vi "conf FCC Main RSE Measurement.vi"(8 "error in (no error)":errorcluster, 11 "SA Measurement in":refnum<class "SA Measurement.lvclass">) -> (0 "error out":errorcluster, 3 "SA Measurement out":refnum<class "SA Measurement.lvclass">)   [LabVIEW 2023, in "Spectrum Analyzer.lvlib" / "SA Measurement.lvclass"]
uses:
  SA Measurement.lvclass
  TYPE DEFINITION/TYPE RBW and VBW Select.ctl
  TYPE DEFINITION/Keysight 9020A/TYPE Measurement Preset.ctl
  SA Measurement.lvclass/SA Measurement.ctl
  Interface_Spectrum/Interface_Spectrum.lvclass
  Spectrum Analyzer.lvlib
  TYPE DEFINITION/TYPE Average Mode Select.ctl
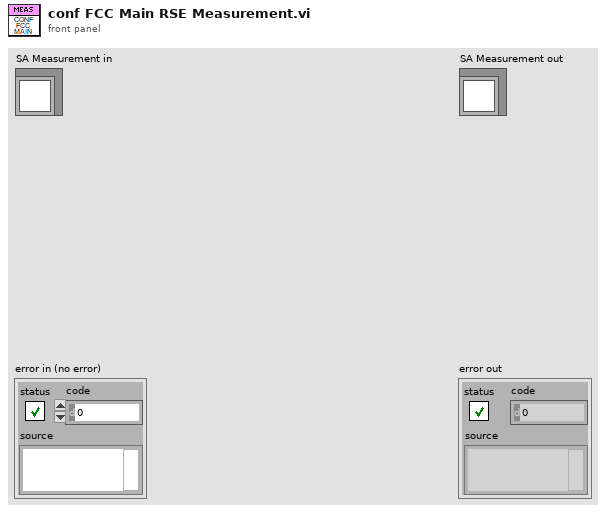
[diagram p1: front panel]
types:
  T1 = typedef "Spectrum Analyzer.lvlib/TYPE Average Mode Select.ctl" = enum16{"Linear(Voltage Avg)", "Video(Log)", "Power"}
  T2 = typedef "Spectrum Analyzer.lvlib/TYPE Measurement Preset.ctl" = enum16{"Sweep SA Mode", "Channel Power", "Occupied BW", "ACP", "Spurious Emission", "Spurious Emission Mask", "Burst Power (Transmit Power)"}
  T3 = typedef "Spectrum Analyzer.lvlib/TYPE RBW and VBW Select.ctl" = enum16{"Res BW", "Video BW"}
  T4 = typedef "Spectrum Analyzer.lvlib/TYPE Y-axis Unit.ctl" = enum16{"dBm", "dBmV", "dBuV", "dBpW", "Volt", "Ampere", "Watt"}
  T5 = typedef "Spectrum Analyzer.lvlib/TYPE Start and Stop Frequency.ctl" = cluster{"Start":dbl, "Stop":dbl}
  T6 = typedef "Spectrum Analyzer.lvlib/TYPE Reference Level and Atten Param.ctl" = cluster{"Reference Level":dbl, "Atten":i32, "Atten Auto?":bool, "Reference Level Offset":dbl}
  T7 = typedef "Spectrum Analyzer.lvlib/TYPE Display Trace Mode Select.ctl" = enum16{"Clear Write", "Max Hold", "Min Hold", "Average", "View"}
  T8 = typedef "Spectrum Analyzer.lvlib/TYPE Detect Mode Select.ctl" = enum16{"Det Auto (Normal)", "Auto Peak", "Positive Peak", "Negative Peak", "Sample", "RMS", "Average", "Quasipeak", "CISPR Average", "RMS Average"}
  T9 = cluster{"Trace Mode":T7, "Detector Type":T8, "Detect Auto?":bool}[]
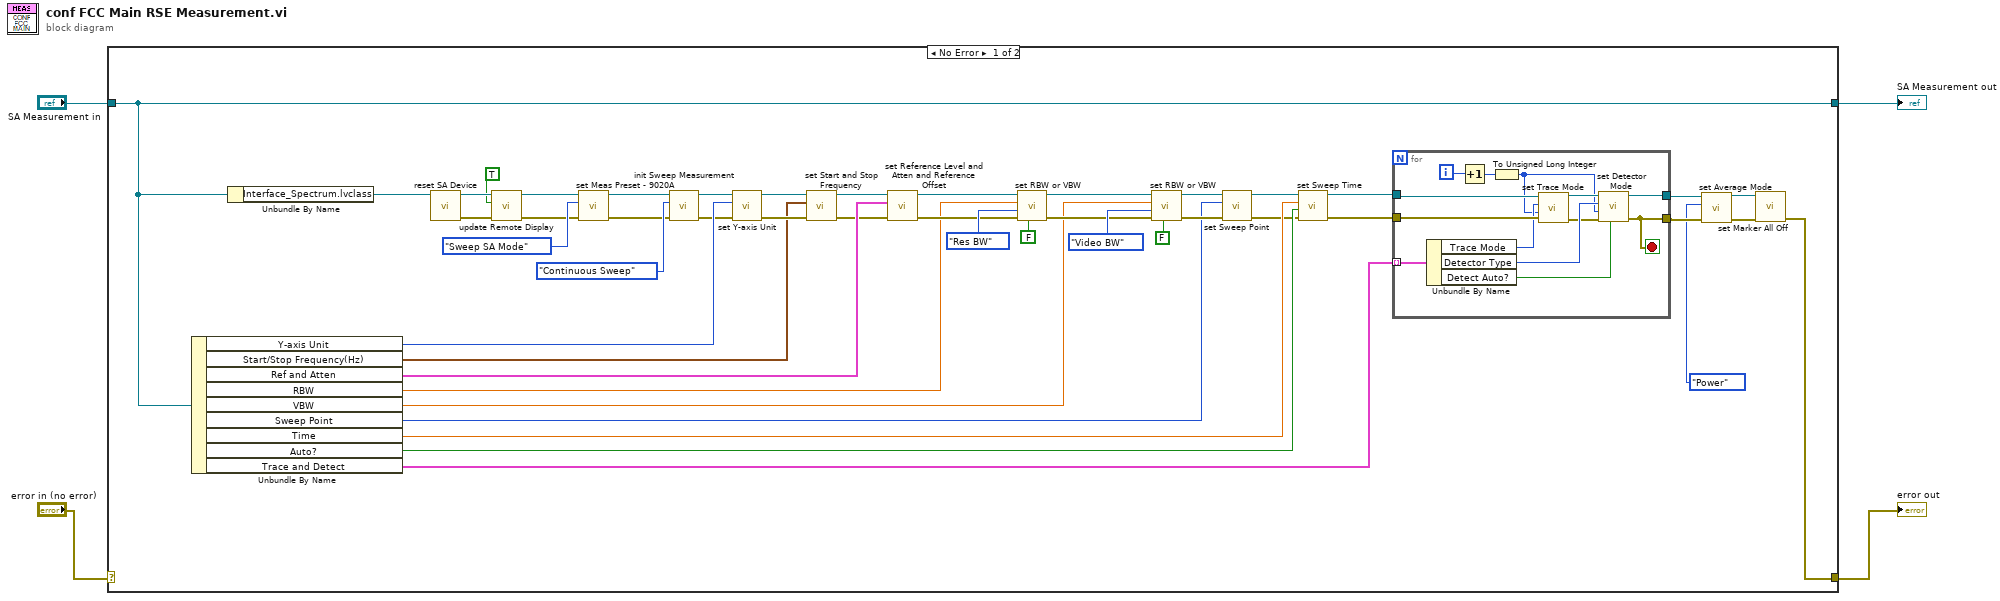
[diagram p0: block diagram]
diagram:
  n1 = case shown="No Error" "error in (no error)" {
    selector: "error in (no error)" -> [_ w65]
    tunnel: [w10 w65] -> w1
    tunnel: [w49 w64] -> w2
    tunnel: "SA Measurement in" -> [w49 w64]
    frame No Error {
      n2 = Unbundle By Name(w49) -> ("Y-axis Unit"=w48:T4, "Start/Stop Frequency(Hz)"=w19:T5, "Ref and Atten"=w41:T6, "RBW"=w38:dbl, "VBW"=w37:dbl, "Sweep Point"=w14:u32, "Time"=w12:dbl, "Auto?"=w36:bool, "Trace and Detect"=w33:T9)
      n3 = Unbundle By Name(w49) -> ("Interface_Spectrum.lvclass"=w50:refnum<class "Interface_Spectrum.lvclass">)
      n4 = call-dynamic "reset SA Device.vi"("Interface_Spectrum in"=w50) -> ("error out"=w31:errorcluster, "Interface_Spectrum out"=w32:refnum<class "Interface_Spectrum.lvclass">)  [unwired: 9 in]
      n5 = call-dynamic "update Remote Display.vi"("error in (no error)"=w31, "Remote Display On?"=TRUE, "Interface_Spectrum in"=w32) -> ("error out"=w24:errorcluster, "Interface_Spectrum out"=w25:refnum<class "Interface_Spectrum.lvclass">)  [unwired: 7 in]
      n6 = call-dynamic "set Meas Preset - 9020A.vi"("error in (no error)"=w24, "Measurement Preset"=TYPE_Measurement_Preset."Sweep SA Mode", "Interface_Spectrum in"=w25) -> ("error out"=w22:errorcluster, "Interface_Spectrum out"=w23:refnum<class "Interface_Spectrum.lvclass">)  [unwired: 7 in]
      n7 = call-dynamic "init Sweep Measurement.vi"("error in (no error)"=w22, "Sweep Measurement Mode"=enum16{"Single Sweep", "Continuous Sweep"}."Continuous Sweep", "Interface_Spectrum in"=w23) -> ("error out"=w27:errorcluster, "Interface_Spectrum out"=w28:refnum<class "Interface_Spectrum.lvclass">)  [unwired: 7 in]
      n8 = call-dynamic "set Y-axis Unit.vi"("error in (no error)"=w27, "Y-axis Unit"=w48, "Interface_Spectrum in"=w28) -> ("error out"=w20:errorcluster, "Interface_Spectrum out"=w21:refnum<class "Interface_Spectrum.lvclass">)  [unwired: 7 in]
      n9 = call-dynamic "set Start and Stop Frequency.vi"("error in (no error)"=w20, "Start/Stop Frequency(Hz)"=w19, "Interface_Spectrum in"=w21) -> ("error out"=w17:errorcluster, "Interface_Spectrum out"=w18:refnum<class "Interface_Spectrum.lvclass">)  [unwired: 7 in]
      n10 = call-dynamic "set Reference Level and Atten and Reference Offset.vi"("error in (no error)"=w17, "Reference Level, Atten, Reference Offset"=w41, "Interface_Spectrum in"=w18) -> ("error out"=w39:errorcluster, "Interface_Spectrum out"=w40:refnum<class "Interface_Spectrum.lvclass">)  [unwired: 7 in]
      n11 = call-dynamic "set RBW or VBW.vi"("BW Auto?"=FALSE, "error in (no error)"=w39, "BW Type"=TYPE_RBW_and_VBW_Select."Res BW", "BW Value (Hz)"=w38, "Interface_Spectrum in"=w40) -> ("error out"=w42:errorcluster, "Interface_Spectrum out"=w43:refnum<class "Interface_Spectrum.lvclass">)  [unwired: 5 in]
      n12 = call-dynamic "set RBW or VBW.vi"("BW Auto?"=FALSE, "error in (no error)"=w42, "BW Type"=TYPE_RBW_and_VBW_Select."Video BW", "BW Value (Hz)"=w37, "Interface_Spectrum in"=w43) -> ("error out"=w15:errorcluster, "Interface_Spectrum out"=w16:refnum<class "Interface_Spectrum.lvclass">)  [unwired: 5 in]
      n13 = call-dynamic "set Sweep Point.vi"("error in (no error)"=w15, "Sweep Point"=w14, "Interface_Spectrum in"=w16) -> ("error out"=w11:errorcluster, "Interface_Spectrum out"=w13:refnum<class "Interface_Spectrum.lvclass">)  [unwired: 7 in]
      n14 = call-dynamic "set Sweep Time.vi"("error in (no error)"=w11, "Sweep Time Auto?"=w36, "Sweep Time(sec)"=w12, "Interface_Spectrum in"=w13) -> ("error out"=w34:errorcluster, "Interface_Spectrum out"=w35:refnum<class "Interface_Spectrum.lvclass">)  [unwired: 6 in]
      n15 = for {
        tunnel: w35 -> [w62]
        tunnel: w34 -> [w61]
        tunnel: w33 -> [w63] mode=indexing
        tunnel: [w51] -> w7
        tunnel: [w52] -> w9
        i -> [w60]
        stop <- w51 stop-if-true
        n16 = Unbundle By Name(w63) -> ("Trace Mode"=w58:T7, "Detector Type"=w56:T8, "Detect Auto?"=w53:bool)
        n17 = Increment(x=w60) -> (x+1=w59:i32)
        n18 = To Unsigned Long Integer(number=w59) -> (unsigned 32bit integer=w54:u32)
        n19 = call-dynamic "set Trace Mode.vi"("error in (no error)"=w61, "Trace Index"=w54, "Trace Mode"=w58, "Interface_Spectrum in"=w62) -> ("error out"=w55:errorcluster, "Interface_Spectrum out"=w57:refnum<class "Interface_Spectrum.lvclass">)  [unwired: 6 in]
        n20 = call-dynamic "set Detector Mode.vi"("Detect Auto?"=w53, "error in (no error)"=w55, "Trace Index"=w54, "Detector Type"=w56, "Interface_Spectrum in"=w57) -> ("error out"=w51:errorcluster, "Interface_Spectrum out"=w52:refnum<class "Interface_Spectrum.lvclass">)  [unwired: 5 in]
      }
      n21 = call-dynamic "set Average Mode.vi"("error in (no error)"=w7, "Average Mode"=TYPE_Average_Mode_Select."Power", "Interface_Spectrum in"=w9) -> ("error out"=w6:errorcluster, "Interface_Spectrum out"=w8:refnum<class "Interface_Spectrum.lvclass">)  [unwired: 7 in]
      n22 = call-dynamic "set Marker All Off.vi"("error in (no error)"=w6, "Interface_Spectrum in"=w8) -> ("error out"=w10:errorcluster)  [unwired: 8 in, 1 out]
    }
    frame Error {
    }
  }
  "error out" <- w1
  "SA Measurement out" <- w2
